vi "Decode Header Value.vi"(11 "value":string) -> (3 "decoded value":string)   [LabVIEW 2020, in "MCP Server.lvlib"]
doc: "Decodes an MCP request header value written as =?base64?...?= (prefix in any case, Base64 or Base64URL), for Check Modern MCP Request.vi. Any other value is returned unchanged."
uses:
  MCP Server.lvlib
  <vilib>/JDP Science/JDP Science Common Utilities/Base64/Base64 Support.lvlib
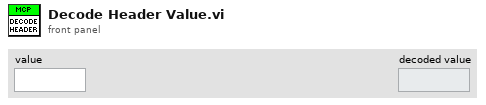
[diagram p1: front panel]
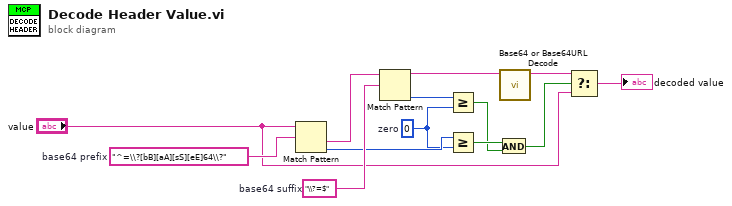
[diagram p0: block diagram]
diagram:
  w8 = 0  # zero
  w11 = "\\?=$"  # base64 suffix
  w13 = "^=\\?[bB][aA][sS][eE]64\\?"  # base64 prefix
  n1 = Match Pattern(string="value", regular expression=w13) -> (after substring=w12:string, offset past match=w10:i32)  [unwired: 1 in, 2 out]
  n2 = Match Pattern(string=w12, regular expression=w11) -> (before substring=w5:string, offset past match=w9:i32)  [unwired: 1 in, 2 out]
  n3 = Greater Or Equal?(x=w9, y=w8) -> (x >= y?=w6:bool)
  n4 = Greater Or Equal?(x=w10, y=w8) -> (x >= y?=w7:bool)
  n5 = And(x=w7, y=w6) -> (x .and. y?=w3:bool)
  n6 = call <vilib>:"Base64 or Base64URL Decode.vi"("Base64 or Base64URL"=w5) -> ("Decoded"=w4:string)  [unwired: 10 in]
  n7 = Select(t=w4, s=w3, f="value") -> (s? t:f=→"decoded value":string)
